vi "BitBlt Wrapper Template.vi"(0 "hdc":u64, 1 "x":i32, 2 "y":i32, 3 "cx":i32, 4 "cy":i32, 5 "hdcSrc":u64, 6 "x1":i32, 7 "y1":i32, 8 "rop":u32=13369376, 9 "error in":errorcluster) -> (20 "return value":i32, 27 "error out":errorcluster)   [LabVIEW 2020]
doc: "Copies the cx x cy pixels at (x1, y1) of the device context hdcSrc to (x, y) of the device context hdc through gdi32.dll BitBlt (stdcall, called in any thread). With hdcSrc = user32 GetDC.vi of a window and rop SRCCOPY (0x00CC0020) this reads the window's client area as Windows composited it last - the window's own redirection surface, so also when it is covered by other windows (measured on Windows 11 with a LabVIEW front panel), without asking the window to draw itself. return value is the Win32 BOOL: non-zero on success, 0 on failure. When error in carries an error the DLL is not called. Generated by tools\\Build Win32 Wrappers.vi - do not edit by hand, rebuild it."
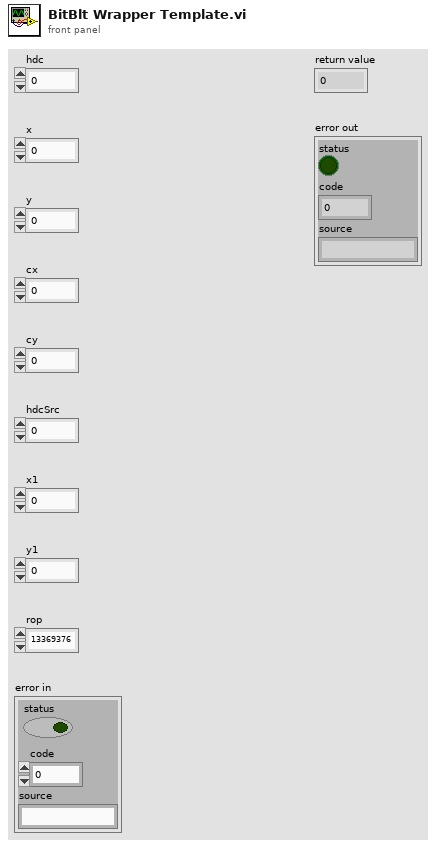
[diagram p1: front panel]
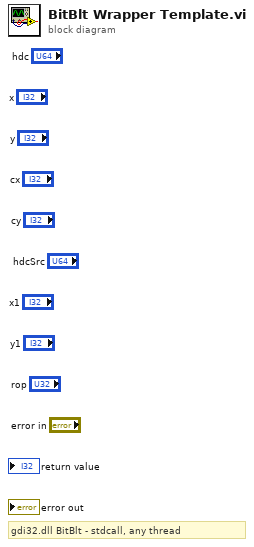
[diagram p0: block diagram]
diagram:
  # "gdi32.dll BitBlt - stdcall, any thread"
